vi "Get Device Info.vi"(8 "error in (no error)":errorcluster, 11 "RIO Device":T1) -> (0 "error out":errorcluster, 1 "SI Channels":string[](array[string]), 2 "SI Count":i32, 3 "Module Name":string)   [LabVIEW 2025, in "I2C Bus Monitor UI.lvlib"]
uses:
  I2C Bus Monitor UI.lvlib
  <vilib>/userDefined/Silver/nirio_resource_slv.ctl
  Error Global.vi
  <vilib>/nisyscfg/Close (Filter).vi
  <vilib>/nisyscfg/Close (System).vi
  <vilib>/nisyscfg/Close (Hardware).vi
  <vilib>/nisyscfg/nisyscfg.lvlib
  <resource>/objmgr/niflexrioatomicsae.rc
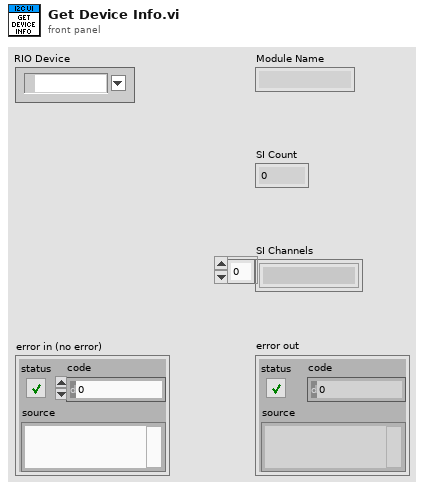
[diagram p1: front panel]
types:
  T1 = typedef "nirio_resource_slv.ctl" = tag
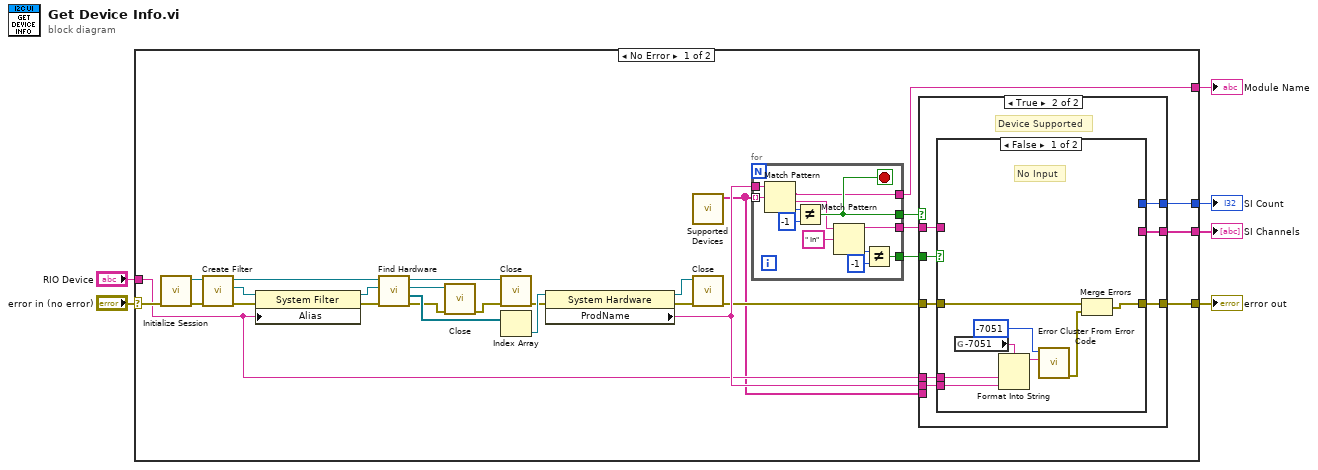
[diagram p0: block diagram]
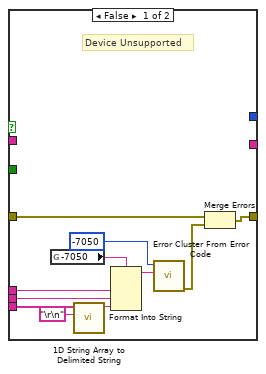
[diagram p2: hidden frame]
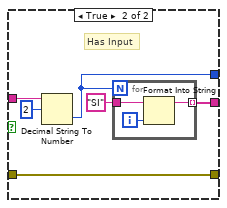
[diagram p3: hidden frame]
diagram:
  n1 = case shown="No Error" "error in (no error)" {
    selector: "error in (no error)" -> [w34 w83]
    tunnel: [w33 _] -> w5
    tunnel: [w32 _] -> w4
    tunnel: [w30 _] -> w3
    tunnel: "RIO Device" -> [w9 _]
    tunnel: [w8 w83] -> w1
    frame No Error {
      n2 = call <vilib>:"Initialize Session.vi"("error in (no error)"=w34) -> ("error out"=w26:errorcluster, "Session out"=w24:refnum<k21>)  [unwired: 9 in]
      n3 = call <vilib>:"Create Filter.vi"("error in (no error)"=w26, "Session in"=w24) -> ("error out"=w21:errorcluster, "Filter out"=w22:refnum<k20>, "Session out"=w25:refnum<k21>)  [unwired: 7 in]
      n4 = property class="System Filter"(reference=w22, error in=w21, "Alias"=w9) -> (reference out=w23:refnum<k20>, error out=w27:errorcluster)
      n5 = call <vilib>:"Find Hardware.vi"("error in (no error)"=w27, "Filter in"=w23, "Session in"=w25) -> ("error out"=w12:errorcluster, "Resources out"=w20:refnum<k20>[], "Filter out"=w11:refnum<k20>, "Session out"=w19:refnum<k21>)  [unwired: 5 in]
      n6 = call-poly <vilib>:"Close.vi"("error in (no error)"=w12, "Filter in"=w11) -> ("error out"=w10:errorcluster)  [unwired: 9 in]
      n7 = call-poly <vilib>:"Close.vi"("error in (no error)"=w10, "Session in"=w19) -> ("error out"=w18:errorcluster)  [unwired: 9 in]
      n8 = Index Array(array=w20) -> (element=w28:refnum<k20>)  [unwired: 1 in]
      n9 = property class="System Hardware"(reference=w28, error in=w18) -> (reference out=w15:refnum<k20>, error out=w14:errorcluster, "ProdName"=w16:string)
      n10 = call "Supported Devices.vi"() -> ("Supported Devices"=w7:string[])  [unwired: 11 in]
      n11 = call-poly <vilib>:"Close.vi"("error in (no error)"=w14, "Resource in"=w15) -> ("error out"=w13:errorcluster)  [unwired: 9 in]
      n12 = for {
        tunnel: w7 -> [w76] mode=indexing
        tunnel: w16 -> [w82]
        tunnel: [w79] -> w17
        tunnel: [w75] -> w32
        tunnel: [w73] -> w29
        tunnel: [w72] -> w31
        stop <- w79 stop-if-true
        n13 = Match Pattern(string=w82, regular expression=w76) -> (match substring=w75:string, after substring=w71:string, offset past match=w81:i32)  [unwired: 1 in, 1 out]
        n14 = Not Equal?(x=w81, y=-1) -> (x != y?=w79:bool)
        n15 = Match Pattern(string=w71, regular expression=" In") -> (before substring=w73:string, offset past match=w77:i32)  [unwired: 1 in, 2 out]
        n16 = Not Equal?(x=w77, y=-1) -> (x != y?=w72:bool)
      }
      n17 = case shown="True" w17 {
        tunnel: [_ w53] -> w33
        tunnel: w31 -> [_ w52]
        tunnel: [_ w51] -> w30
        tunnel: w29 -> [_ w50]
        tunnel: w13 -> [w39 w49]
        tunnel: [w38 w48] -> w8
        tunnel: w16 -> [w36 w47]
        tunnel: w7 -> [w44 _]
        tunnel: w9 -> [w35 w46]
        frame False {
          # "Device Unsupported"
          n18 = global read "Error Global.vi" "-7050"() -> (w45:string)
          n19 = call <vilib>:"1D String Array to Delimited String.vi"("delimiter"="\r\n", "string array"=w44) -> ("delimited string"=w42:string)  [unwired: 9 in]
          n20 = Format Into String(format string=w45, w35, w36, w42) -> (resulting string=w41:string)  [unwired: 2 in, 1 out]
          n21 = call <vilib>:"Error Cluster From Error Code.vi"("error message (\"\")"=w41, "error code (0)"=-7050) -> ("error out"=w37:errorcluster)  [unwired: 7 in]
          n22 = Merge Errors(w39, w37) -> (w38:errorcluster)
        }
        frame True {
          # "Device Supported"
          n23 = case shown="False" w52 {
            tunnel: w50 -> [_ w67]
            tunnel: [_ w65] -> w53
            tunnel: [_ w63] -> w51
            tunnel: w49 -> [w57 w62]
            tunnel: [w56 w62] -> w48
            tunnel: w47 -> [w55 _]
            tunnel: w46 -> [w54 _]
            frame False {
              # "No Input"
              n24 = global read "Error Global.vi" "-7051"() -> (w61:string)
              n25 = Format Into String(format string=w61, w54, w55) -> (resulting string=w60:string)  [unwired: 2 in, 1 out]
              n26 = call <vilib>:"Error Cluster From Error Code.vi"("error message (\"\")"=w60, "error code (0)"=-7051) -> ("error out"=w58:errorcluster)  [unwired: 7 in]
              n27 = Merge Errors(w57, w58) -> (w56:errorcluster)
            }
            frame True {
              # "Has Input"
              n28 = Decimal String To Number(string=w67, offset=2) -> (number=w65:i32)  [unwired: 1 in, 1 out]
              n29 = for {
                N: w65 -> [_]
                tunnel: "SI" -> [w70]
                tunnel: [w68] -> w63 mode=indexing
                i -> [w69]
                n30 = Format Into String(initial string=w70, w69) -> (resulting string=w68:string)  [unwired: 2 in, 1 out]
              }
            }
          }
        }
      }
    }
    frame Error {
    }
  }
  "SI Count" <- w5
  "Module Name" <- w4
  "SI Channels" <- w3
  "error out" <- w1
